vi "RDB Receive.vi"(8 "error in (no error)":errorcluster, 10 "RDB Reference in":T4, 11 "Settings":T1={"UDP Receiver"=refnum, "UDP Sender"=refnum, "Valid Packet"=FALSE, "TCP"=refnum, "Network Settings"={"IP adress"="127.0.0.1", "RDB"={"Protocol"=enum."UDP", "Tx Port"=48270, "Rx Port"=10, "Buffer Size"=204800, "Timeout"=10}, "SCP"={"Protocol"=enum."TCP", "Tx Port"=48191, "Rx Port"=48191, "Buffer Size"=204800, "Timeout"=10}}, "vclient"=path "", "paeseHandle"=0, "builderHandle"=0}) -> (0 "error out":errorcluster, 2 "RDB Reference out":T4, 3 "Settings":T1={"UDP Receiver"=refnum, "UDP Sender"=refnum, "Valid Packet"=FALSE, "TCP"=refnum, "Network Settings"={"IP adress"="127.0.0.1", "RDB"={"Protocol"=enum."UDP", "Tx Port"=48270, "Rx Port"=10, "Buffer Size"=204800, "Timeout"=10}, "SCP"={"Protocol"=enum."TCP", "Tx Port"=48191, "Rx Port"=48191, "Buffer Size"=204800, "Timeout"=10}}, "vclient"=path "", "paeseHandle"=0, "builderHandle"=0})   [LabVIEW 2023, in "RDB.lvlib"]
uses:
  RDB.lvlib
  RDB References.ctl
  DataContainer/DataContainer.lvclass
  Engine/Type/Settings.ctl
  Shared/Network Settings.ctl
  Shared/Protocol.ctl
  Engine/Vires VTD Engine.lvlib
  Shared/Vires VTD Shared.lvlib
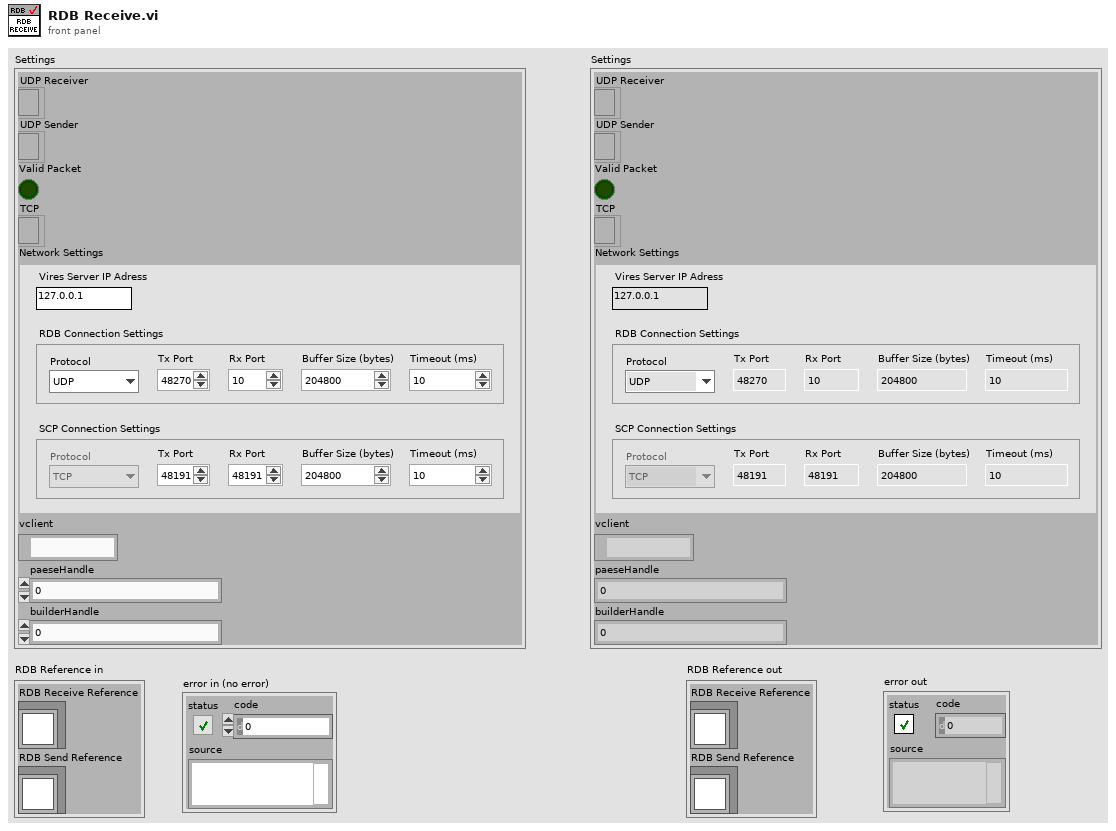
[diagram p1: front panel]
types:
  T1 = typedef "Vires VTD Engine.lvlib/Settings.ctl" = cluster{"UDP Receiver":refnum<k16>, "UDP Sender":refnum<k16>, "Valid Packet":bool, "TCP":refnum<k5>, "Network Settings":T2, "vclient":path, "paeseHandle":u64, "builderHandle":u64}
  T2 = typedef "Vires VTD Shared.lvlib/Network Settings.ctl" = cluster{"IP adress":string, "RDB":cluster{"Protocol":T3, "Tx Port":u16, "Rx Port":u16, "Buffer Size":i32, "Timeout":u16}, "SCP":cluster{"Protocol":T3, "Tx Port":u16, "Rx Port":u16, "Buffer Size":i32, "Timeout":u16}}
  T3 = typedef "Vires VTD Shared.lvlib/Protocol.ctl" = enum16{"UDP", "TCP"}
  T4 = typedef "RDB.lvlib/RDB References.ctl" = cluster{"RDB Receive Reference":refnum<class "DataContainer.lvclass">, "RDB Send Reference":refnum<class "DataContainer.lvclass">}
  T5 = typedef "XNET Frame FlexRay.ctl" = cluster{"timestamp":timestamp, "payload":u8[], "slot":u16, "type":T6, "cycle count":u8, "startup?":bool, "sync?":bool, "preamble?":bool, "ch A":bool, "ch B":bool, "echo?":bool}
  T6 = typedef "XNET Frame Type FlexRay.ctl" = u8
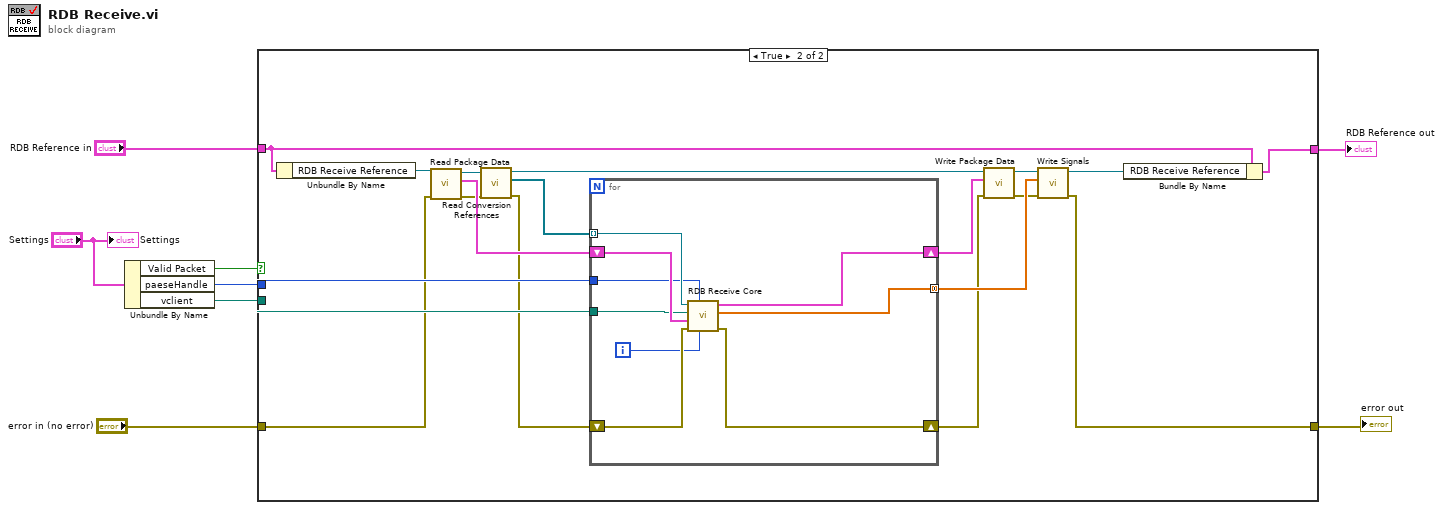
[diagram p0: block diagram]
diagram:
  n1 = Unbundle By Name("Settings") -> ("Valid Packet"=w2:bool, "paeseHandle"=w1:u64, "vclient"=w3:path)
  n2 = case shown="True" w2 {
    tunnel: "RDB Reference in" -> [w10 w26]
    tunnel: [w10 w29] -> w7
    tunnel: "error in (no error)" -> [w9 w17]
    tunnel: [w9 w11] -> w5
    tunnel: w3 -> [_ w28]
    tunnel: w1 -> [_ w27]
    frame False {
    }
    frame True {
      n3 = Unbundle By Name(w26) -> ("RDB Receive Reference"=w25:refnum<class "DataContainer.lvclass">)
      n4 = call-dynamic "Read Package Data.vi"("error in (no error)"=w17, "DataContainer in"=w25) -> ("error out"=w16:errorcluster, "Package Data"=w23:T5[], "DataContainer out"=w24:refnum<class "DataContainer.lvclass">)  [unwired: 7 in]
      n5 = call-dynamic "Read Conversion References.vi"("error in (no error)"=w16, "DataContainer in"=w24) -> ("error out"=w15:errorcluster, "Conversion References"=w22:refnum<k21>[], "DataContainer out"=w19:refnum<class "DataContainer.lvclass">)  [unwired: 7 in]
      n6 = for {
        shift-right: [w34] -> w14
        shift-left: w15 -> [w38]
        tunnel: w22 -> [w35] mode=indexing
        shift-right: [w36] -> w21
        shift-left: w23 -> [w37]
        tunnel: [w33] -> w20 mode=concatenating
        tunnel: w28 -> [w32]
        tunnel: w27 -> [w30]
        i -> [w31]
        n7 = call "RDB Receive Core.vi"("index"=w31, "paeseHandle in"=w30, "error in (no error)"=w38, "RDB Data in"=w37, "vclient"=w32, "XNET Conversion"=w35) -> ("error out"=w34:errorcluster, "signal data"=w33:dbl[], "RDB Data out"=w36:T5[])  [unwired: 3 in]
      }
      n8 = call-dynamic "Write Package Data.vi"("error in (no error)"=w14, "Package Data"=w21, "DataContainer in"=w19) -> ("error out"=w13:errorcluster, "DataContainer out"=w18:refnum<class "DataContainer.lvclass">)  [unwired: 7 in]
      n9 = call-dynamic "Write Signals.vi"("error in (no error)"=w13, "Signals"=w20, "DataContainer in"=w18) -> ("error out"=w11:errorcluster, "DataContainer out"=w12:refnum<class "DataContainer.lvclass">)  [unwired: 7 in]
      n10 = Bundle By Name(cluster=w26, "RDB Receive Reference"=w12) -> (w29:T4)
    }
  }
  "RDB Reference out" <- w7
  "error out" <- w5
  "Settings" <- "Settings"
